vi "onCreate.vi"(8 "error in (no error)":errorcluster, 11 "Server in":refnum<class "Server.lvclass">) -> (0 "error out":errorcluster, 3 "Server out":refnum<class "Server.lvclass">)   [LabVIEW 2013, in "MQTT Server.lvlib" / "Server.lvclass"]
uses:
  Server.lvclass
  SessionRef -- cluster.ctl
  <vilib>/LabVIEW Open Source Project/MQTT Connection/MQTT_Base/Base Class/Response -- cluster.ctl
  <vilib>/LabVIEW Open Source Project/MQTT Control Packets/Control Packets/ControlPacket/ControlPacket.lvclass
  Subscription/_Subscription.lvclass
  Private Events -- cluster.ctl
  <vilib>/LabVIEW Open Source Project/MQTT Control Packets/Control Packets/PUBLISH/PUBLISH.lvclass
  <vilib>/LabVIEW Open Source Project/MQTT Control Packets/Control Packets/Ack/Ack.lvclass
  Statistics -- cluster.ctl
  <vilib>/LabVIEW Open Source Project/MQTT Connection/MQTT_Base/Base Class/MQTT_Base.lvclass
  Server.lvclass/Server.ctl
  StoredSessions/StoredSessions.lvclass
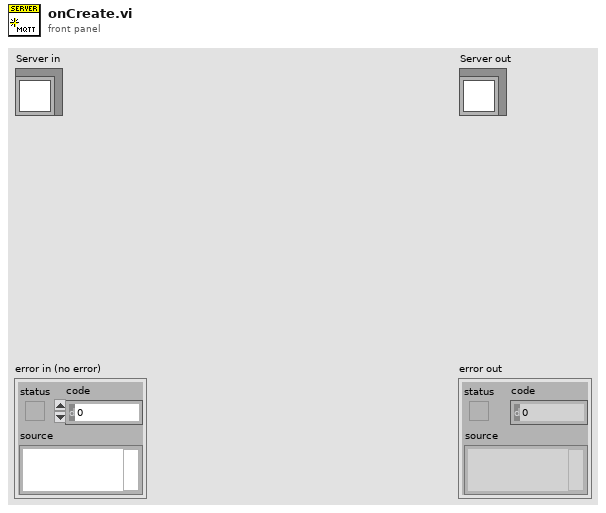
[diagram p1: front panel]
types:
  T1 = typedef "MQTT Server.lvlib/Server.lvclass/Statistics -- cluster.ctl" = cluster{"Nb Connections":u32, "Nb Subscriptions":u32}
  T2 = typedef "MQTT Server.lvlib/Server.lvclass/Private Events -- cluster.ctl" = cluster{"Inbound Packet":refnum<user-event>, "Inbound Ack":refnum<user-event>}
  T3 = typedef "MQTT Server.lvlib/Server.lvclass/SessionRef -- cluster.ctl" = cluster{"ClientID":string, "SessionMailbox":refnum<queue>}
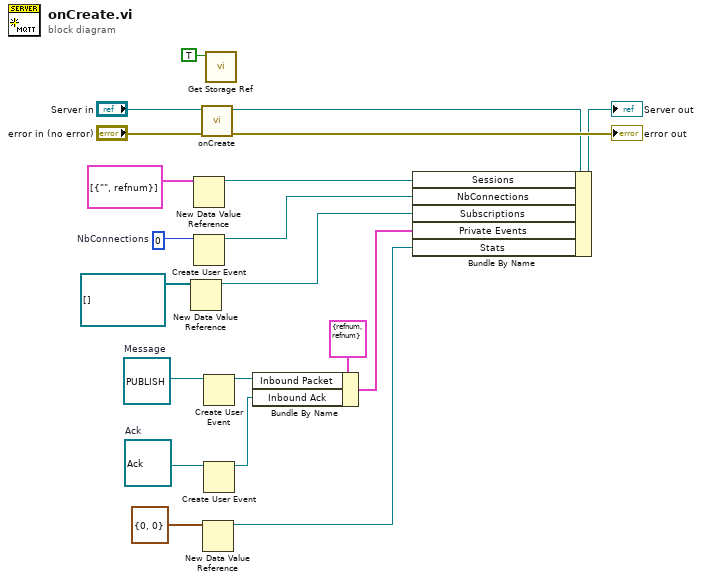
[diagram p0: block diagram]
diagram:
  w5 = refnum<class "Ack.lvclass"> refnum  # Ack
  w6 = refnum<class "PUBLISH.lvclass"> refnum  # Message
  w14 = u32 0  # NbConnections
  n1 = New Data Value Reference(data value=refnum<class "_Subscription.lvclass">[] []) -> (data value reference=w9:refnum<data-value>)  [unwired: 1 in, 1 out]
  n2 = New Data Value Reference(data value=T3[] [{"ClientID"="", "SessionMailbox"=refnum}]) -> (data value reference=w16:refnum<data-value>)  [unwired: 1 in, 1 out]
  n3 = Create User Event(user event datatype=w14) -> (user event=w13:refnum<user-event>)  [unwired: 1 in, 1 out]
  n4 = call-parent "onCreate.vi"("error in (no error)"="error in (no error)", "MQTT_Base in"="Server in") -> ("error out"=→"error out":errorcluster, "MQTT_Base out"=w15:refnum<class "Server.lvclass">)  [unwired: 8 in]
  n5 = New Data Value Reference(data value=T1 {"Nb Connections"=0, "Nb Subscriptions"=0} ("Statistics")) -> (data value reference=w1:refnum<data-value>)  [unwired: 1 in, 1 out]
  n6 = Create User Event(user event datatype=w6) -> (user event=w7:refnum<user-event>)  [unwired: 1 in, 1 out]
  n7 = Create User Event(user event datatype=w5) -> (user event=w4:refnum<user-event>)  [unwired: 1 in, 1 out]
  n8 = call "Get Storage Ref.vi"("Init (F)"=TRUE) -> ()  [unwired: 10 in, 1 out]
  n9 = Bundle By Name(cluster=T2 {"Inbound Packet"=refnum, "Inbound Ack"=refnum} ("Private Events"), "Inbound Packet"=w7, "Inbound Ack"=w4) -> (w3:T2)
  n10 = Bundle By Name(cluster=w15, "Sessions"=w16, "NbConnections"=w13, "Subscriptions"=w9, "Private Events"=w3, "Stats"=w1) -> (→"Server out":refnum<class "Server.lvclass">)
